vi "IsIconic Wrapper Template.vi"(0 "hWnd":u64, 11 "error in":errorcluster) -> (4 "minimized?":bool, 15 "error out":errorcluster)   [LabVIEW 2020]
doc: "TRUE when the window hWnd is minimized (iconic), through user32.dll IsIconic (stdcall, called in any thread). FALSE also when hWnd is not a window. When error in carries an error the DLL is not called. Generated by tools\\Build Win32 Wrappers.vi - do not edit by hand, rebuild it."
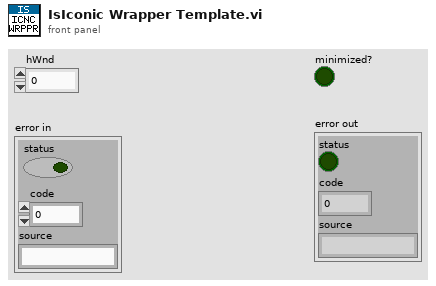
[diagram p1: front panel]
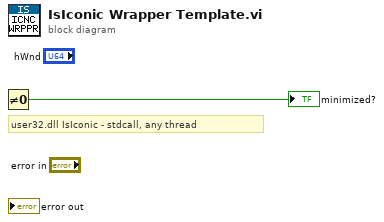
[diagram p0: block diagram]
diagram:
  # "user32.dll IsIconic - stdcall, any thread"
  n1 = Not Equal To 0?() -> (x != 0?=→"minimized?":bool)  [unwired: 1 in]
